vi "Run_All_Caraya.vi"() -> ()   [LabVIEW 2026]
doc: "Caraya suite runner, generated by lvai_generate_caraya_test_runner.\n\nIt builds every test VI's path relative to its OWN location, so the suite moves with the folder, and runs them through Caraya's Run Tests.vi (Array Path instance) with Interactive FALSE - a TRUE there opens a modal report dialog, which stops LabVIEW's gRPC service until a human dismisses it.\n\nRead the JUnit report named by 'Report Path used', not 'error out': the error cluster carries the FIRST failed assertion only."
uses:
  <vilib>/addons/_JKI Toolkits/Caraya/run-tests/Run Test (Array Path).vi
  <vilib>/addons/_JKI Toolkits/Caraya/Caraya.lvlib
panel:
  out "error out":errorcluster
  out "Report Path used":path
  in  "error in":errorcluster
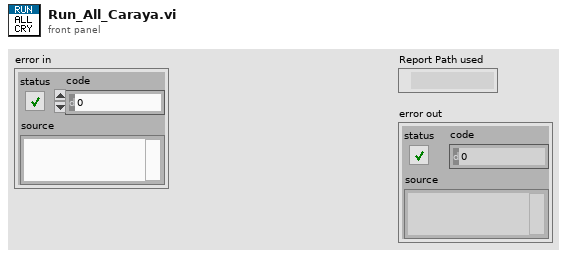
[diagram p1: front panel]
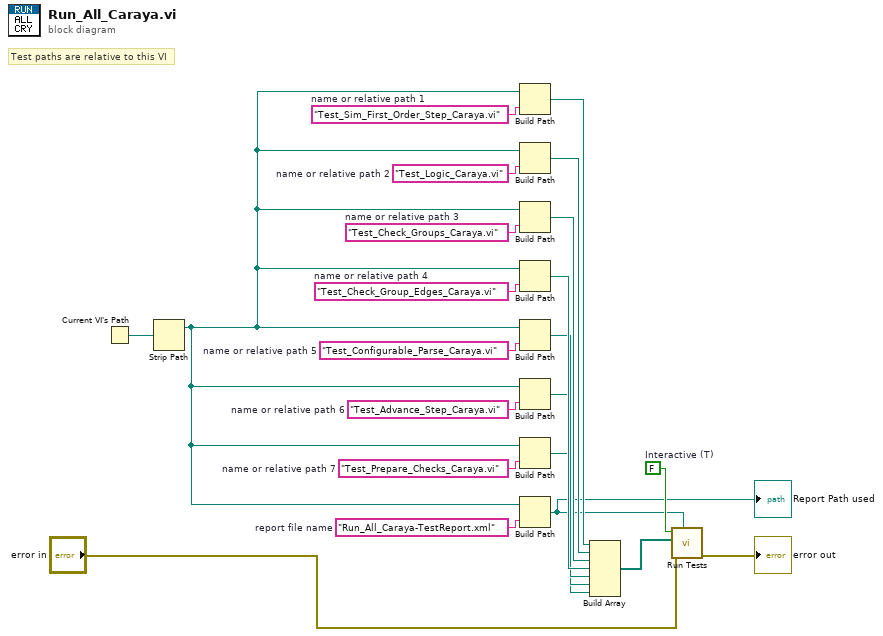
[diagram p0: block diagram]
diagram:
  w5 = FALSE  # Interactive (T)
  w13 = "Run_All_Caraya-TestReport.xml"  # report file name
  w15 = "Test_Prepare_Checks_Caraya.vi"  # name or relative path 7
  w16 = "Test_Advance_Step_Caraya.vi"  # name or relative path 6
  w17 = "Test_Configurable_Parse_Caraya.vi"  # name or relative path 5
  w18 = "Test_Check_Group_Edges_Caraya.vi"  # name or relative path 4
  w19 = "Test_Check_Groups_Caraya.vi"  # name or relative path 3
  w20 = "Test_Logic_Caraya.vi"  # name or relative path 2
  w21 = "Test_Sim_First_Order_Step_Caraya.vi"  # name or relative path 1
  # "Test paths are relative to this VI"
  n1 = Current VI's Path() -> (path=w22:path)
  n2 = Strip Path(path=w22) -> (stripped path=w14:path)  [unwired: 1 out]
  n3 = Build Path(base path=w14, name or relative path=w21) -> (appended path=w12:path)
  n4 = Build Path(base path=w14, name or relative path=w20) -> (appended path=w11:path)
  n5 = Build Path(base path=w14, name or relative path=w19) -> (appended path=w10:path)
  n6 = Build Path(base path=w14, name or relative path=w18) -> (appended path=w9:path)
  n7 = Build Path(base path=w14, name or relative path=w17) -> (appended path=w8:path)
  n8 = Build Path(base path=w14, name or relative path=w16) -> (appended path=w7:path)
  n9 = Build Path(base path=w14, name or relative path=w15) -> (appended path=w6:path)
  n10 = Build Path(base path=w14, name or relative path=w13) -> (appended path=w2:path)
  "Report Path used" <- w2
  n11 = Build Array(w12, w11, w10, w9, w8, w7, w6) -> (w4:path[])
  n12 = call-poly <vilib>:"Run Tests.vi"("Report Path"=w2, "error in"="error in", "Paths"=w4, "Interactive (T)"=w5) -> ("error out"=→"error out":errorcluster)  [unwired: 6 in, 1 out]
